vi "RFH-convert-r140andLibreVNA.vi"() -> ()   [LabVIEW 2020, in "RFH-Reflection_File_Handler.lvlib"]
doc: "Run by hand: converts the R140 Excel files and the LibreVNA files of a measurement folder to the common format and verifies them. The user picks the main folder, the subfolders and the frequency range."
uses:
  RFH-Reflection_File_Handler.lvlib
panel:
  out "LibreVNA":T1(graph)
  out "Ref":T1(graph)
  out "Frequency":dbl[][](graph)
  in  "Max Frequency (6G)":dbl=6000000000.0 format="%#_13p"
  in  "Min Frequency  (0.2G)":dbl=200000000.0 format="%#_13p"
  out "All Good libreVNA?":bool
  out "All Good ref?":bool
  out "All OK?":bool
  in  "Convertion Folder":string="Converted Data"
  in  "LibreVNA file folder":string="LibreVNA"
  in  "ref excel file folder":string="R140"
  in  "Measurement Main Folder":path
  out "error out LibreVNA":errorcluster
  out "error out ref":errorcluster
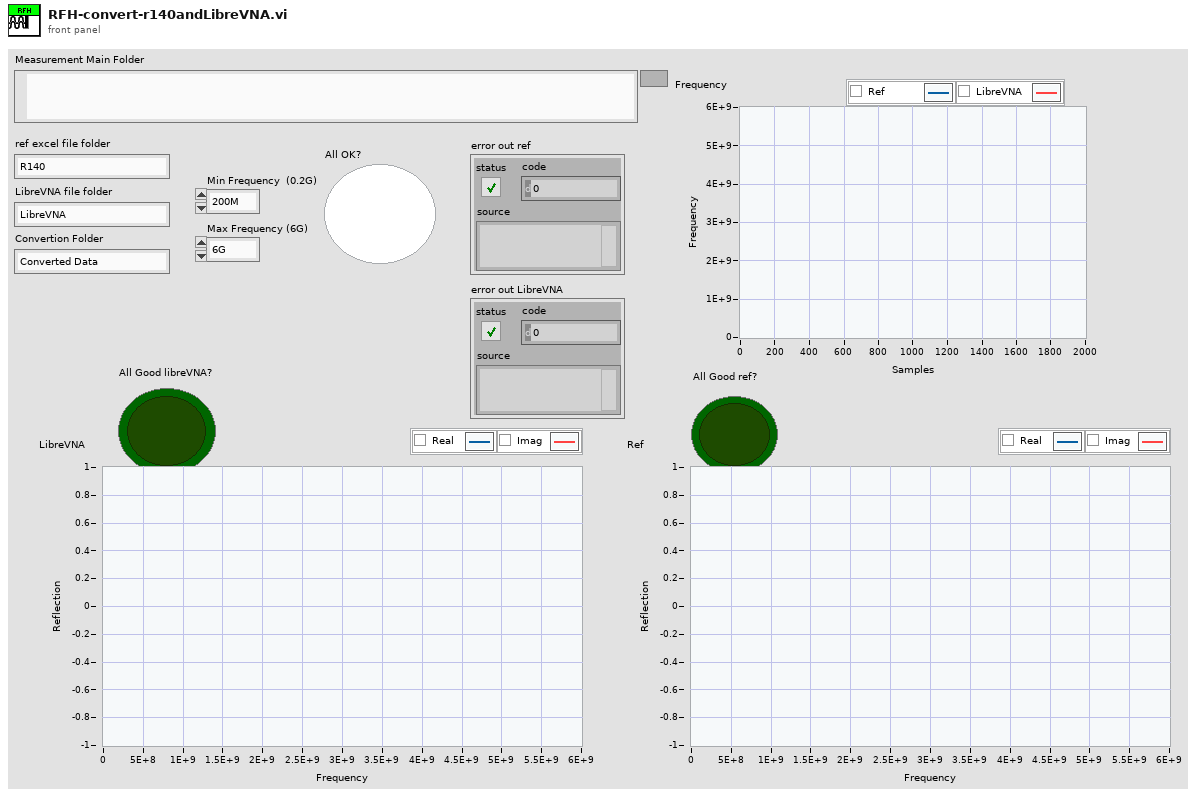
[diagram p1: front panel]
types:
  T1 = cluster{"Frequency":dbl[], "Reflection''":dbl[]}[]
  T2 = typedef "RFH-Reflection_File_Handler.lvlib/RFH-common_data_format.ctl" = cluster{"Frequency":dbl[], "Reflection'":dbl[], "Reflection''":dbl[], "Permativity'":dbl[], "Permativity''":dbl[], "Conductivity":dbl[], "Loss Tangent":dbl[], "Resistance":dbl[], "Reactance":dbl[]}
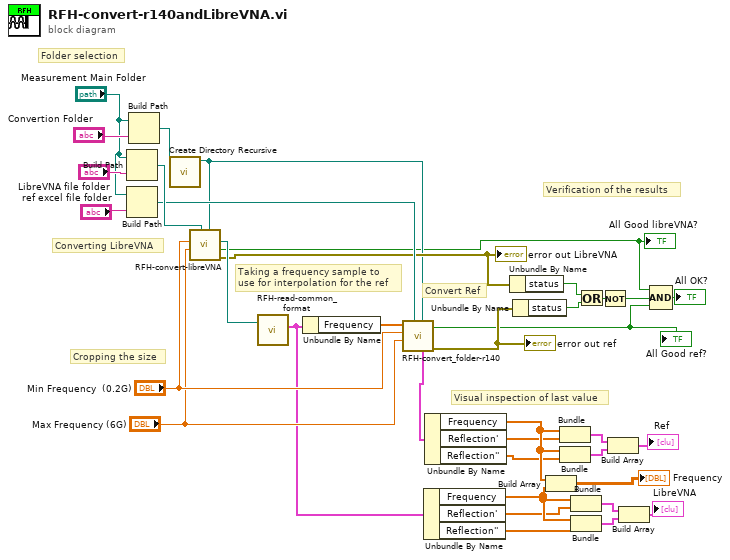
[diagram p0: block diagram]
diagram:
  # "Convert Ref"
  # "Taking a frequency sample to\nuse for interpolation for the ref"
  # "Converting LibreVNA"
  # "Verification of the results"
  # "Folder selection"
  # "Cropping the size"
  # "Visual inspection of last value"
  n1 = Build Path(base path="Measurement Main Folder", name or relative path="LibreVNA file folder") -> (appended path=w34:path)
  n2 = Build Path(base path="Measurement Main Folder", name or relative path="ref excel file folder") -> (appended path=w29:path)
  n3 = Build Path(base path="Measurement Main Folder", name or relative path="Convertion Folder") -> (appended path=w23:path)
  n4 = call <vilib>:"Create Directory Recursive.vi"("directory"=w23) -> ("directory copy"=w22:path)  [unwired: 4 in, 2 out]
  n5 = call "RFH-convert-libreVNA.vi"("destionation path"=w22, "All libreVNA data folder"=w34, "Max Frequency (6G)"="Max Frequency (6G)", "Min Frequency  (0.3G)"="Min Frequency  (0.2G)") -> ("error out"=w28:errorcluster, "All Good?"=w18:bool, "last file"=w30:path)  [unwired: 4 in, 1 out]
  "error out LibreVNA" <- w28
  "All Good libreVNA?" <- w18
  n6 = call "RFH-read-common_format.vi"("file path (dialog if empty)"=w30) -> ("Common Format"=w15:T2)  [unwired: 9 in, 1 out]
  n7 = Unbundle By Name(w15) -> ("Frequency"=w36:dbl[])
  n8 = call "RFH-convert_folder-r140.vi"("Destination Folder"=w22, "Folder Path"=w29, "Max Frequency (6G)"="Max Frequency (6G)", "Min Frequency  (0.3G)"="Min Frequency  (0.2G)", "Xi"=w36) -> ("error out"=w27:errorcluster, "All Good?"=w19:bool, "Last Value"=w14:T2)  [unwired: 4 in]
  "error out ref" <- w27
  "All Good ref?" <- w19
  n9 = Unbundle By Name(w15) -> ("Frequency"=w12:dbl[], "Reflection'"=w11:dbl[], "Reflection''"=w10:dbl[])
  n10 = Unbundle By Name(w14) -> ("Frequency"=w4:dbl[], "Reflection'"=w3:dbl[], "Reflection''"=w2:dbl[])
  n11 = Unbundle By Name(w28) -> ("status"=w26:bool)
  n12 = Unbundle By Name(w27) -> ("status"=w25:bool)
  n13 = Build Array(w4, w12) -> (→"Frequency":dbl[][])
  n14 = Bundle("Frequency"=w4, "Reflection'"=w3) -> (w5:cluster{"Frequency":dbl[], "Reflection'":dbl[]})  [unwired: 1 in]
  n15 = Bundle("Frequency"=w4, "Reflection''"=w2) -> (w6:cluster{"Frequency":dbl[], "Reflection''":dbl[]})  [unwired: 1 in]
  n16 = Bundle("Frequency"=w12, "Reflection'"=w11) -> (w9:cluster{"Frequency":dbl[], "Reflection'":dbl[]})  [unwired: 1 in]
  n17 = Bundle("Frequency"=w12, "Reflection''"=w10) -> (w8:cluster{"Frequency":dbl[], "Reflection''":dbl[]})  [unwired: 1 in]
  n18 = Or(x=w26, y=w25) -> (x .or. y?=w24:bool)
  n19 = Not(x=w24) -> (.not. x?=w17:bool)
  n20 = Build Array(w5, w6) -> (→"Ref":T1)
  n21 = Build Array(w9, w8) -> (→"LibreVNA":T1)
  n22 = Compound Arithmetic op=AND(w18, w17, w19) -> (→"All OK?":bool)
